vi "Read SM.vi"(8 "error in (no error)":errorcluster, 10 "Vo":dbl, 11 "Puerto serial":refnum<visa-resource-name>) -> (0 "error out":errorcluster, 3 "Acquistion Data":T1)   [LabVIEW 2020]
uses:
  39de7056-9ed4-47ec-a934-0fe14cb6d8de.vi
  68284e2b-69f7-4644-8932-20630b6eccd7.vi
  controls/Acquisition data --typedef.ctl
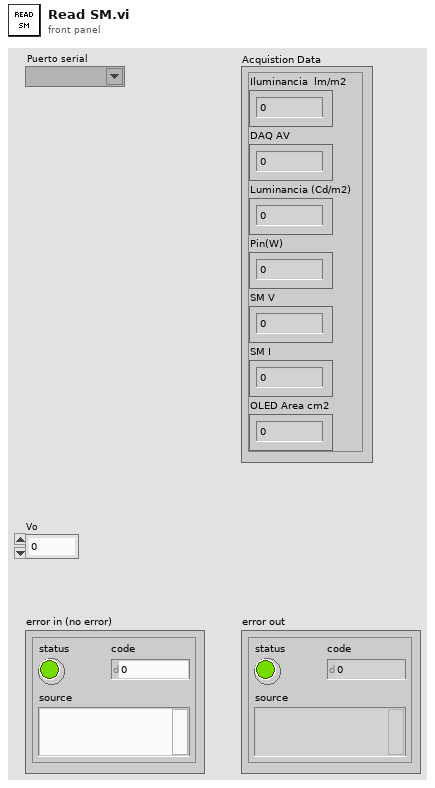
[diagram p1: front panel]
types:
  T1 = typedef "Acquisition data --typedef.ctl" = cluster{"Iluminancia  lm/m2":dbl, "DAQ AV":dbl, "Luminancia (Cd/m2)":dbl, "Pin(W)":dbl, "SM V":dbl, "SM I":dbl, "OLED Area cm2":dbl}
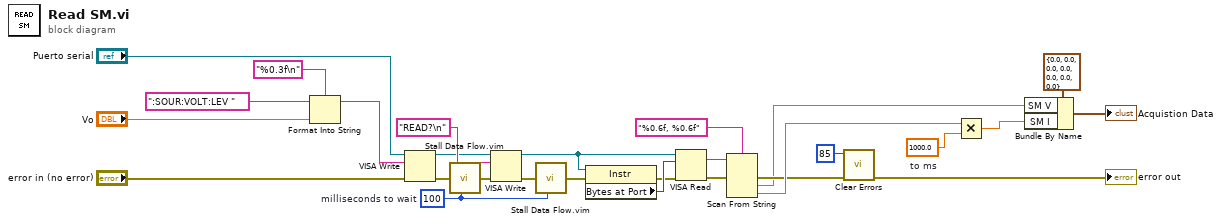
[diagram p0: block diagram]
diagram:
  w12 = 1000.0  # to ms
  w3 = u32 100  # milliseconds to wait
  n1 = Format Into String(format string="%0.3f\n", initial string=":SOUR:VOLT:LEV " ("Comando"), "Vo") -> (resulting string=w4:string)  [unwired: 1 in, 1 out]
  n2 = VISA Write(VISA resource name="Puerto serial", write buffer=w4, error in (no error)="error in (no error)") -> (VISA resource name out=w21:refnum<visa-resource-name>, error out=w20:errorcluster)  [unwired: 1 out]
  n3 = call "Stall Data Flow.vim"("value in"=w20, "milliseconds to wait"=w3) -> ("value out"=w22:errorcluster)  [unwired: 1 out]
  n4 = VISA Write(VISA resource name=w21, write buffer="READ?\n" ("Comando"), error in (no error)=w22) -> (VISA resource name out=w27:refnum<visa-resource-name>, error out=w23:errorcluster)  [unwired: 1 out]
  n5 = call "Stall Data Flow.vim"("value in"=w23, "milliseconds to wait"=w3) -> ("value out"=w24:errorcluster)  [unwired: 1 out]
  n6 = property class="Instr"(reference=w27, error in=w24) -> (error out=w26:errorcluster, "Bytes at Port"=w28:u32)  [unwired: 1 out]
  n7 = VISA Read(VISA resource name=w27, byte count=w28, error in (no error)=w26) -> (read buffer=w16:string, error out=w17:errorcluster)  [unwired: 2 out]
  n8 = Scan From String(format string="%0.6f, %0.6f", input string=w16, error in=w17) -> (error out=w13:errorcluster, output 1=w10:dbl, output 2=w14:dbl)  [unwired: 3 in, 2 out]
  n9 = call <vilib>:"Clear Errors.vi"("error in (no error)"=w13, "specific error code to clear (0: all)"=85) -> ("error out"=→"error out":errorcluster)  [unwired: 4 in, 1 out]
  n10 = Multiply(x=w14, y=w12) -> (x*y=w9:dbl)
  n11 = Bundle By Name(cluster=T1 {"Iluminancia  lm/m2"=0.0, "DAQ AV"=0.0, "Luminancia (Cd/m2)"=0.0, "Pin(W)"=0.0, "SM V"=0.0, "SM I"=0.0, "OLED Area cm2"=0.0} ("Acquistion Data"), "SM V"=w10, "SM I"=w9) -> (→"Acquistion Data":T1)
